vi "showOCRResultwithBB.vi"(4 "BB Color":u32(colorbox)=16711680, 5 "Font, Size & Style":T1={"Desired Font (Application)"=enum."Application Font", "[User-specified Font]"={"Font Name"="", "Size"=12, "Strikeout?"=FALSE, "Italic?"=FALSE, "Underline?"=FALSE, "Outline?"=FALSE, "Shadow?"=FALSE, "Bold?"=FALSE, "Rotation Angle"=0.0}, "Horizontal Alignment"=0, "Vertical Alignment"=0} {"Vertical Alignment" items=["Bottom", "Top", "Baseline"]; "Horizontal Alignment" items=["Left", "Center", "Right"]; "[User-specified Font]"."Rotation Angle" format="%.2f"}, 6 "drawBB":enum16{"no", "yes"}(ring), 7 "Text Color":u32(colorbox), 8 "error in":errorcluster, 9 "Array":T3[](array[typedef]), 10 "chars":u8[](array[numeric]), 11 "Image in":T2) -> (0 "error out":errorcluster, 3 "Image out":T2)   [LabVIEW 2025, in "adsOCR.lvlib" / "ocr.lvclass"]
doc: "Testing only: support 1 image"
uses:
  ocr.lvclass
  TextDecRecResult2L.ctl
  <vilib>/vision/Image Controls.llb/IMAQ Image.ctl
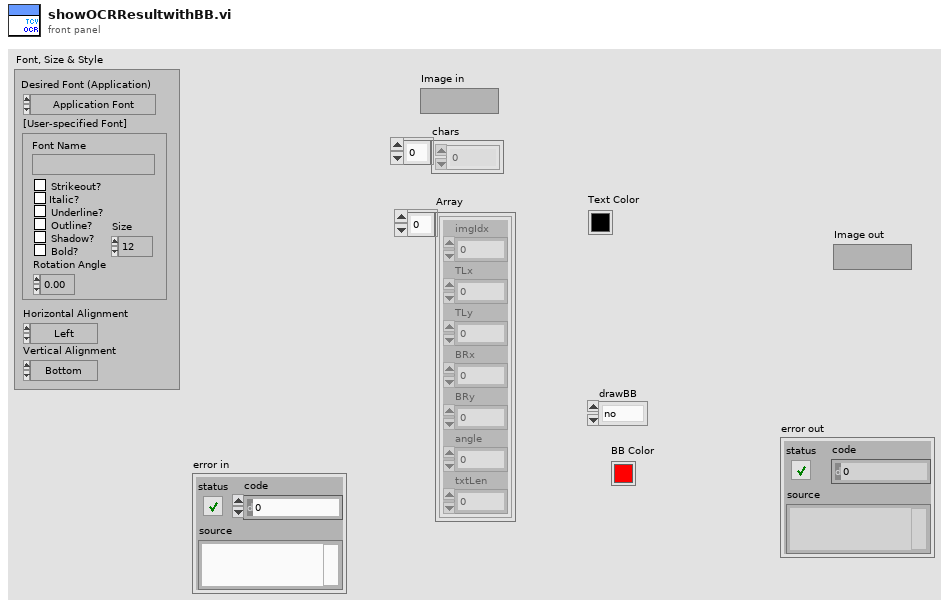
[diagram p1: front panel]
types:
  T1 = cluster{"Desired Font (Application)":enum16{"User-specified Font", "Application Font", "System Font", "Dialog Font"}, "[User-specified Font]":cluster{"Font Name":string, "Size":i16, "Strikeout?":bool, "Italic?":bool, "Underline?":bool, "Outline?":bool, "Shadow?":bool, "Bold?":bool, "Rotation Angle":dbl}, "Horizontal Alignment":i16, "Vertical Alignment":i16}
  T2 = typedef "IMAQ Image.ctl" = refnum<image>
  T3 = typedef "adsOCR.lvlib/ocr.lvclass/TextDecRecResult2L.ctl" = cluster{"imgIdx":i32, "TLx":i32, "TLy":i32, "BRx":i32, "BRy":i32, "angle":sgl, "txtLen":i32}
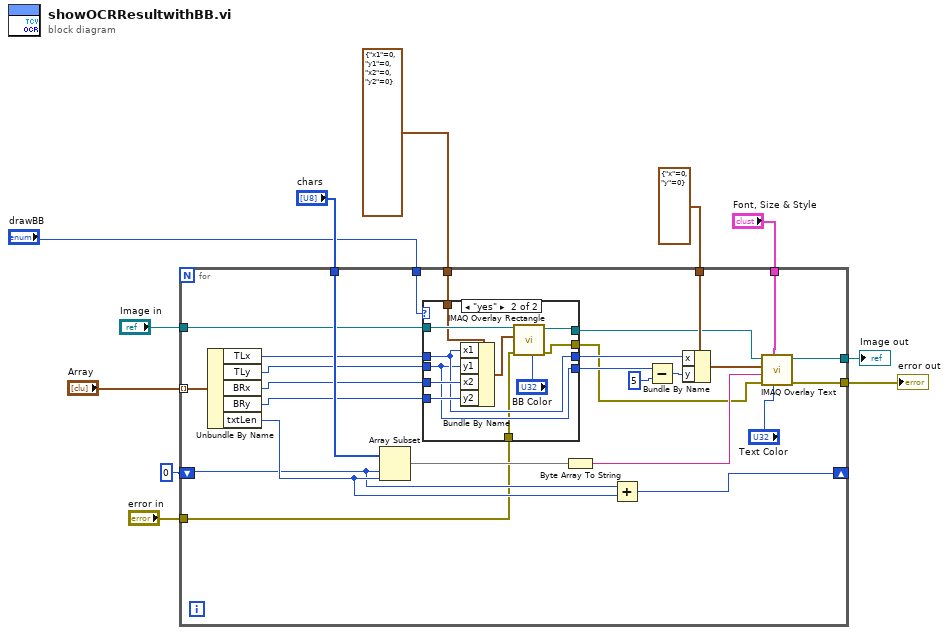
[diagram p0: block diagram]
diagram:
  n1 = for {
    tunnel: "Array" -> [w38] mode=indexing
    tunnel: cluster{"x":i32, "y":i32} {"x"=0, "y"=0} -> [w36]
    tunnel: "Image in" -> [w25]
    shift-right: [w32] -> _
    shift-left: 0 -> [w30]
    tunnel: "chars" -> [w33]
    tunnel: [w27] -> w4
    tunnel: "error in" -> [w16]
    tunnel: [w26] -> w6
    tunnel: cluster{"x1":i32, "y1":i32, "x2":i32, "y2":i32} {"x1"=0, "y1"=0, "x2"=0, "y2"=0} -> [w23]
    tunnel: "drawBB" -> [w14]
    tunnel: "Font, Size & Style" -> [w12]
    n2 = Unbundle By Name(w38) -> ("TLx"=w22:i32, "TLy"=w21:i32, "BRx"=w20:i32, "BRy"=w19:i32, "txtLen"=w31:i32)
    n3 = Array Subset(array=w33, index=w30, length=w31) -> (w29:u8[])
    n4 = case shown="\"yes\"" w14 {
      tunnel: w25 -> [w42 w53]
      tunnel: [w42 w52] -> w24
      tunnel: w23 -> [_ w51]
      tunnel: w22 -> [w41 w47]
      tunnel: w21 -> [w40 w46]
      tunnel: w20 -> [_ w50]
      tunnel: w19 -> [_ w49]
      tunnel: [w41 w47] -> w18
      tunnel: [w40 w46] -> w17
      tunnel: w16 -> [w39 w45]
      tunnel: [w39 w44] -> w15
      frame "no", Default {
      }
      frame "yes" {
        n5 = Bundle By Name(cluster=w51, "x1"=w47, "y1"=w46, "x2"=w50, "y2"=w49) -> (w48:cluster{"x1":i32, "y1":i32, "x2":i32, "y2":i32})
        n6 = call "IMAQ Overlay Rectangle"("Color"="BB Color", "error in (no error)"=w45, "Rectangle"=w48, "Image"=w53) -> ("error out"=w44:errorcluster, "Image Out"=w52:T2)  [unwired: 6 in]
      }
    }
    n7 = Byte Array To String(unsigned byte array=w29) -> (string=w28:string)
    n8 = Add(x=w30, y=w31) -> (x+y=w32:i32)
    n9 = Subtract(x=w17, y=5) -> (x-y=w35:i32)
    n10 = Bundle By Name(cluster=w36, "x"=w18, "y"=w35) -> (w34:cluster{"x":i32, "y":i32})
    n11 = call "IMAQ Overlay Text"("Text Color (black)"="Text Color", "Font, Size & Style"=w12, "error in (no error)"=w15, "String"=w28, "Origin"=w34, "Image"=w24) -> ("error out"=w26:errorcluster, "Image Out"=w27:T2)  [unwired: 4 in]
  }
  "error out" <- w6
  "Image out" <- w4
